vi "Table Buffer - Enqueue.vi"(8 "error in (no error)":errorcluster, 11 "Data":string[][](array[string])) -> (0 "error out":errorcluster, 3 "Overflow":bool)   [LabVIEW 2025, in "I2C Bus Monitor UI.lvlib"]
uses:
  I2C Bus Monitor UI.lvlib
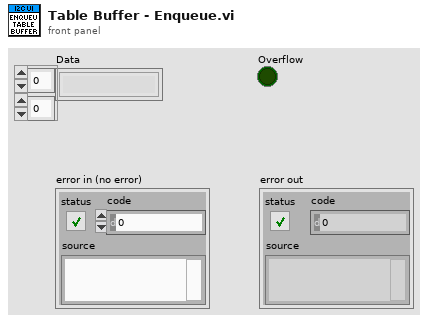
[diagram p1: front panel]
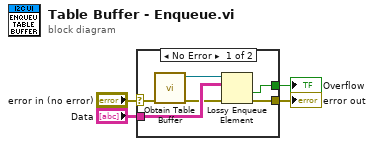
[diagram p0: block diagram]
diagram:
  n1 = case shown="No Error" "error in (no error)" {
    selector: "error in (no error)" -> [w10 w11]
    tunnel: [w9 w11] -> w3
    tunnel: "Data" -> [w8 _]
    tunnel: [w5 _] -> w1
    frame No Error {
      n2 = call "Obtain Table Buffer.vi"("error in (no error)"=w10) -> ("error out"=w6:errorcluster, "Table Queue"=w7:refnum<queue>)  [unwired: 9 in]
      n3 = Lossy Enqueue Element(queue=w7, element=w8, error in (no error)=w6) -> (overflow?=w5:bool, error out=w9:errorcluster)  [unwired: 2 out]
    }
    frame Error {
    }
  }
  "error out" <- w3
  "Overflow" <- w1
